vi "query Marker Value.vi"(8 "error in (no error)":errorcluster, 10 "Marker Index":i32=1 min=1, 11 "FSV-40N in":refnum<class "FSV-40N.lvclass">) -> (0 "error out":errorcluster, 2 "Marker Value":T1 {"X-axis" format="%#_6p"}, 3 "FSV-40N out":refnum<class "FSV-40N.lvclass">)   [LabVIEW 2023, in "Spectrum Analyzer.lvlib" / "FSV-40N.lvclass"]
uses:
  FSV-40N.lvclass
  TYPE DEFINITION/TYPE Marker Value.ctl
  FSV-40N.lvclass/FSV-40N.ctl
  Spectrum Analyzer.lvlib
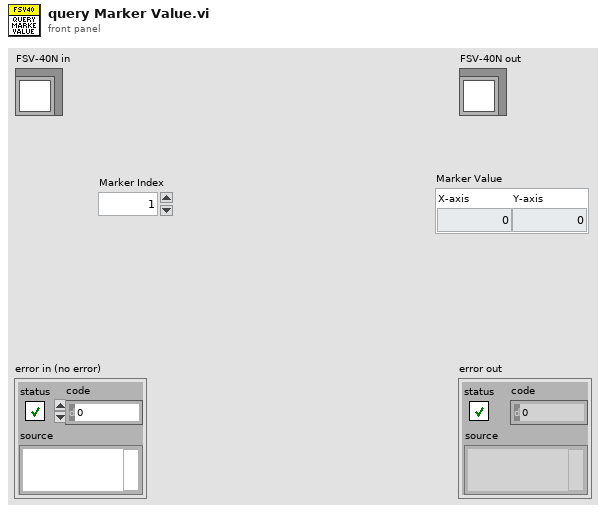
[diagram p1: front panel]
types:
  T1 = typedef "Spectrum Analyzer.lvlib/TYPE Marker Value.ctl" = cluster{"X-axis":dbl, "Y-axis":dbl}
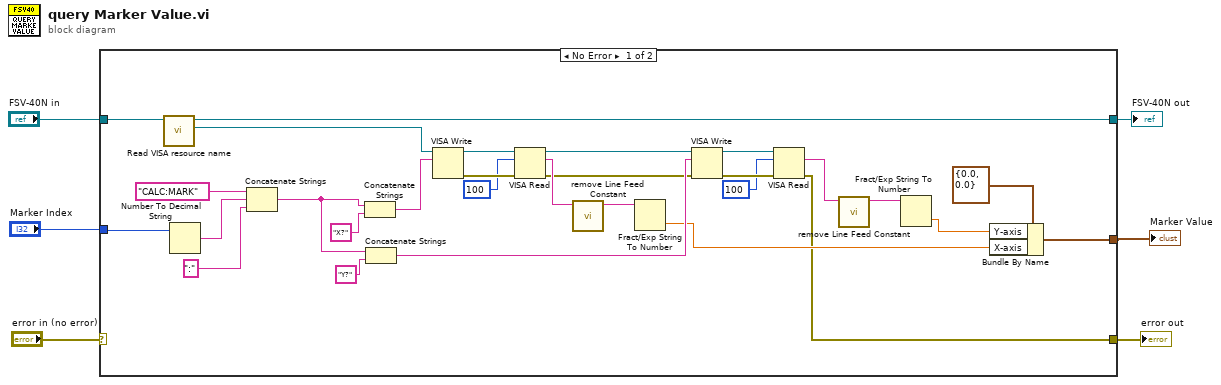
[diagram p0: block diagram]
diagram:
  n1 = case shown="No Error" "error in (no error)" {
    selector: "error in (no error)" -> [_ w36]
    tunnel: "FSV-40N in" -> [w35 w37]
    tunnel: [w9 w37] -> w4
    tunnel: [w7 w36] -> w3
    tunnel: "Marker Index" -> [w34 _]
    tunnel: [w10 _] -> w1
    frame No Error {
      n2 = call "Read VISA resource name.vi"("FSV-40N in"=w35) -> ("VISA resource name"=w30:refnum<visa-resource-name>, "FSV-40N out"=w9:refnum<class "FSV-40N.lvclass">)  [unwired: 8 in, 1 out]
      n3 = Number To Decimal String(number=w34) -> (decimal integer string=w32:string)  [unwired: 1 in]
      n4 = Concatenate Strings("CALC:MARK" ("string"), w32, ":" ("string")) -> (w18:string)
      n5 = Concatenate Strings(w18, "X?" ("string")) -> (w29:string)
      n6 = Concatenate Strings(w18, "Y?" ("string")) -> (w16:string)
      n7 = VISA Write(VISA resource name=w30, write buffer=w29) -> (VISA resource name out=w28:refnum<visa-resource-name>, error out=w27:errorcluster)  [unwired: 1 in, 1 out]
      n8 = VISA Read(VISA resource name=w28, byte count=u32 100, error in (no error)=w27) -> (VISA resource name out=w20:refnum<visa-resource-name>, read buffer=w25:string, error out=w8:errorcluster)  [unwired: 1 out]
      n9 = call "remove Line Feed Constant.vi"("Input String"=w25) -> ("Line Feed Removed String"=w24:string)  [unwired: 10 in]
      n10 = Fract/Exp String To Number(string=w24) -> (number=w11:dbl)  [unwired: 3 in, 1 out]
      n11 = VISA Write(VISA resource name=w20, write buffer=w16, error in (no error)=w8) -> (VISA resource name out=w23:refnum<visa-resource-name>, error out=w22:errorcluster)  [unwired: 1 out]
      n12 = VISA Read(VISA resource name=w23, byte count=u32 100, error in (no error)=w22) -> (read buffer=w14:string, error out=w7:errorcluster)  [unwired: 2 out]
      n13 = call "remove Line Feed Constant.vi"("Input String"=w14) -> ("Line Feed Removed String"=w15:string)  [unwired: 10 in]
      n14 = Fract/Exp String To Number(string=w15) -> (number=w12:dbl)  [unwired: 3 in, 1 out]
      n15 = Bundle By Name(cluster=T1 {"X-axis"=0.0, "Y-axis"=0.0} ("Marker Value 2"), "Y-axis"=w12, "X-axis"=w11) -> (w10:T1)
    }
    frame Error {
    }
  }
  "error out" <- w3
  "FSV-40N out" <- w4
  "Marker Value" <- w1
